vi "Is Error Code.vi"(7 "error in (no error)":errorcluster) -> (2 "code":i32, 3 "Code!=0":bool)   [LabVIEW 2019, in "Error Generation.lvlib"]
doc: "Check if code is unequal ZERO.\n- - -\nCopyright (c) 2023, Merecs Engineering GmbH"
uses:
  Error Generation.lvlib
panel:
  # "Connector Pane"
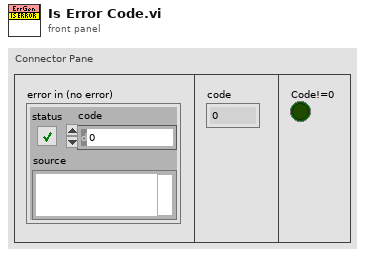
[diagram p1: front panel]
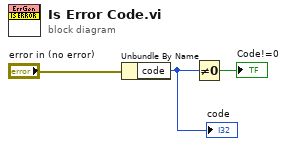
[diagram p0: block diagram]
diagram:
  n1 = Unbundle By Name("error in (no error)") -> ("code"=w2:i32)
  "code" <- w2
  n2 = Not Equal To 0?(x=w2) -> (x != 0?=→"Code!=0":bool)
